vi "VIH Utility - STR - C-Style Escaped String - Build.vi"(5 "Escape codes 80..FF (F)":bool, 7 "Escape space char (T)":bool=TRUE, 10 "Extra characters to escape (none)":string, 11 "String in":string) -> (3 "String out":string)   [LabVIEW 2014]
doc: "::: VI Helpeks :::\nCopyright (c) 2000-2026 Konstantin Shifershteyn. All rights reserved."
panel:
  # "VI Helpeks\nCopyright (c) 2012-2026 Konstantin Shifershteyn"
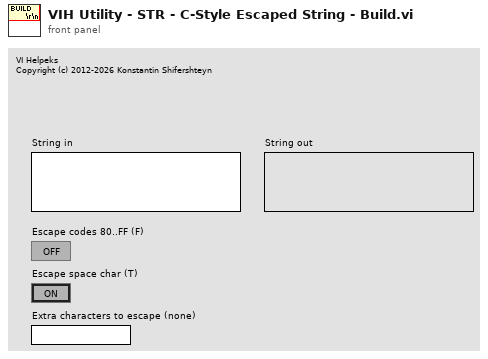
[diagram p1: front panel]
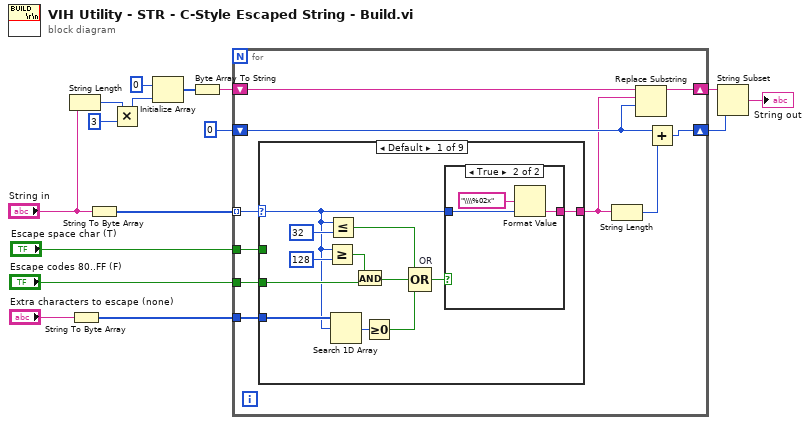
[diagram p0: block diagram]
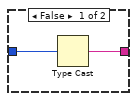
[diagram p2: hidden frame]
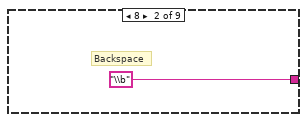
[diagram p3: hidden frame]
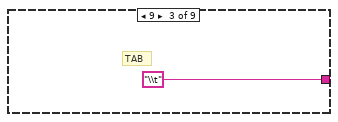
[diagram p4: hidden frame]
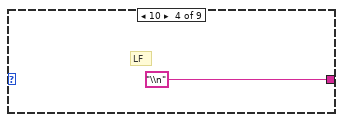
[diagram p5: hidden frame]
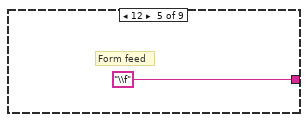
[diagram p6: hidden frame]
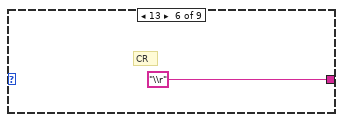
[diagram p7: hidden frame]
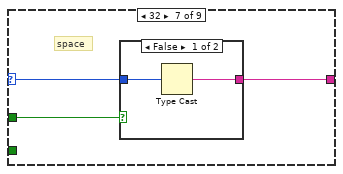
[diagram p8: hidden frame]
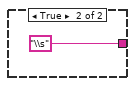
[diagram p9: hidden frame]
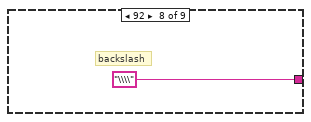
[diagram p10: hidden frame]
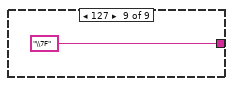
[diagram p11: hidden frame]
diagram:
  n1 = String Length(string="String in") -> (length=w12:i32)
  n2 = String To Byte Array(string="Extra characters to escape (none)") -> (unsigned byte array=w2:u8[])
  n3 = String To Byte Array(string="String in") -> (unsigned byte array=w14:u8[])
  n4 = Multiply(x=w12, y=3) -> (x*y=w10:i32)
  n5 = Initialize Array(u8 0, w10) -> (w9:u8[])
  n6 = Byte Array To String(unsigned byte array=w9) -> (string=w8:string)
  n7 = for {
    tunnel: w14 -> [w26] mode=indexing
    shift-right: [w24] -> w6
    shift-left: w8 -> [w25]
    shift-right: [w22] -> w5
    shift-left: 0 -> [w23]
    tunnel: "Escape codes 80..FF (F)" -> [w19]
    tunnel: w2 -> [w18]
    tunnel: "Escape space char (T)" -> [w17]
    n8 = case shown="Default" w26 {
      selector: w26 -> [w32 _ _ _ _ _ w49 _ _]
      tunnel: [w38 "\\b" ("output string") "\\t" ("output string") "\\n" ("output string") "\\f" ("output string") "\\r" ("output string") w51 "\\\\" ("output string") "\\7F" ("output string")] -> w21
      tunnel: w19 -> [w34 _ _ _ _ _ _ _ _]
      tunnel: w18 -> [w33 _ _ _ _ _ _ _ _]
      tunnel: w17 -> [_ _ _ _ _ _ w50 _ _]
      frame Default {
        n9 = Greater Or Equal?(x=w32, y=u8 128) -> (x >= y?=w35:bool)
        n10 = Less Or Equal?(x=w32, y=u8 32) -> (x <= y?=w28:bool)
        n11 = Search 1D Array(1D array=w33, element=w32) -> (index of element=w31:i32)  [unwired: 1 in]
        n12 = And(x=w35, y=w34) -> (x .and. y?=w30:bool)
        n13 = Greater Or Equal To 0?(x=w31) -> (x >= 0?=w29:bool)
        n14 = Compound Arithmetic op=OR "OR"(w28, w30, w29) -> (w27:bool)
        n15 = case shown="True" w27 {
          tunnel: [w39 w42] -> w38
          tunnel: w32 -> [w40 w41]
          frame False {
            n16 = Type Cast(x=w40) -> (*(type *) &x=w39:string)  [unwired: 1 in]
          }
          frame True {
            n17 = Format Value(format string="\\\\%02x", value (0)=w41) -> (output string=w42:string)  [unwired: 1 in]
          }
        }
      }
      frame 8 {
        # "Backspace"
      }
      frame 9 {
        # "TAB"
      }
      frame 10 {
        # "LF"
      }
      frame 12 {
        # "Form feed"
      }
      frame 13 {
        # "CR"
      }
      frame 32 {
        # "space"
        n18 = case shown="False" w50 {
          tunnel: [w52 "\\s" ("output string")] -> w51
          tunnel: w49 -> [w53 _]
          frame False {
            n19 = Type Cast(x=w53) -> (*(type *) &x=w52:string)  [unwired: 1 in]
          }
          frame True {
          }
        }
      }
      frame 92 {
        # "backslash"
      }
      frame 127 {
      }
    }
    n20 = String Length(string=w21) -> (length=w20:i32)
    n21 = Replace Substring(3:w23, 4:w21, 5:w25) -> (1:w24:string)  [unwired: 1 in, 1 out]
    n22 = Add(x=w23, y=w20) -> (x+y=w22:i32)
  }
  n23 = String Subset(string=w6, length (rest)=w5) -> (substring=→"String out":string)  [unwired: 1 in]
